vi "elevator_v1_working.vi"() -> ()   [LabVIEW 2020]
uses:
  State_enum.ctl
panel:
  in  "Stop Button":bool
  in  "1":bool
  in  "2":bool
  in  "3":bool
  out "Elevator":i8(slide) scale=0.0..10.0
  out "state":T1
  out "Destination floor":i32
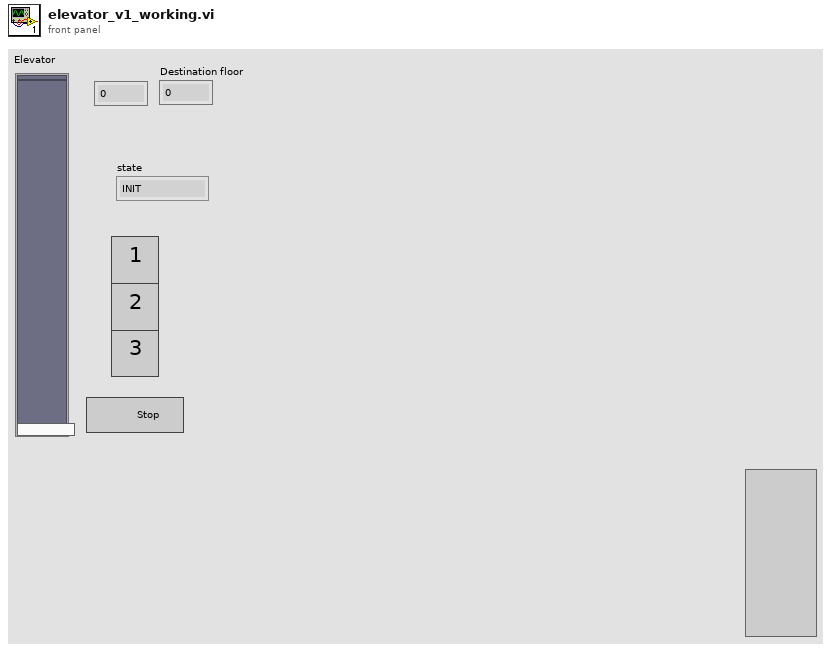
[diagram p1: front panel]
types:
  T1 = typedef "State_enum.ctl" = enum16{"INIT", "ATTENTE", "DEPLACEMENT", "PORTE_OUVERTE", "PORTE_FERMEE", "ARRET_URGENCE"}
  T2 = typedef "State_enum.ctl" = enum16{"Stopped", "Floor1", "Floor2", "Floor3"}
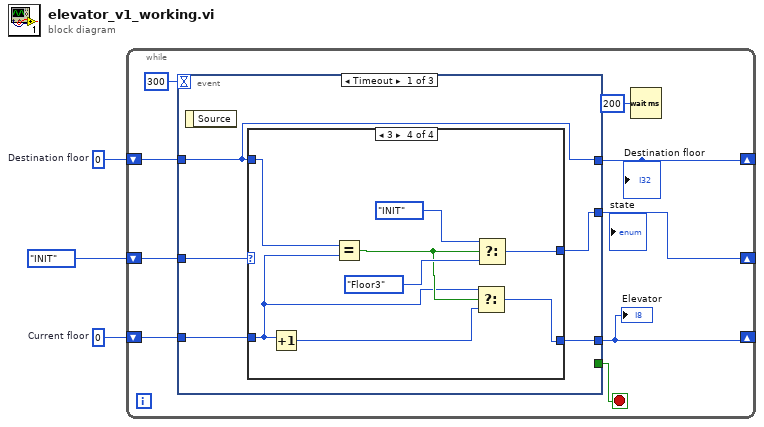
[diagram p0: block diagram]
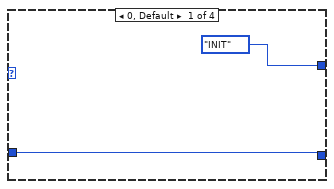
[diagram p2: hidden frame]
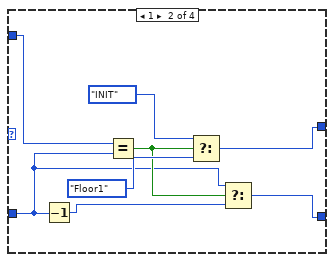
[diagram p3: hidden frame]
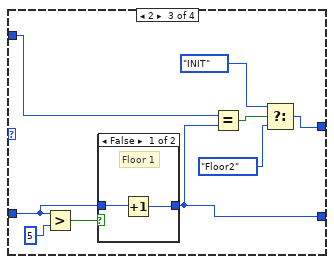
[diagram p4: hidden frame]
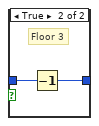
[diagram p5: hidden frame]
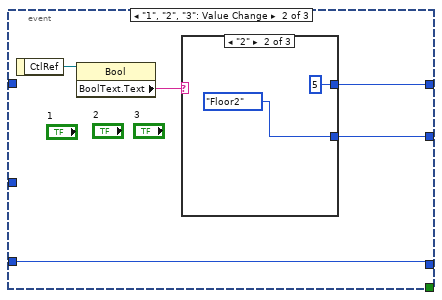
[diagram p6: hidden frame]
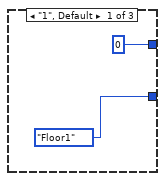
[diagram p7: hidden frame]
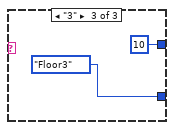
[diagram p8: hidden frame]
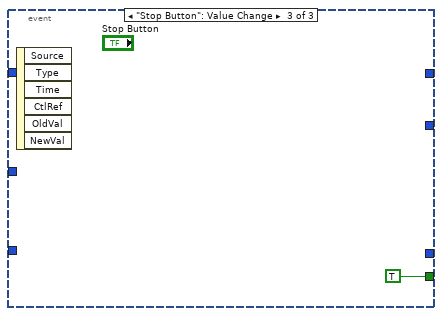
[diagram p9: hidden frame]
diagram:
  w2 = 0  # Current floor
  w3 = 0  # Destination floor
  n1 = while {
    shift-right: [w6] -> _
    shift-left: w3 -> [w7]
    shift-right: [w5] -> _
    shift-left: w2 -> [w9]
    shift-right: [w8] -> _
    shift-left: State_enum."INIT" ("state") -> [w10]
    stop <- w12 stop-if-true
    n2 = event shown="[0] Timeout" {
      selector: _ -> [_ _ _]
      dyn-events: _ -> [_ _ _]
      timeout: 300 -> [_ _ _]
      tunnel: [_ _ TRUE] -> w12
      tunnel: [w13 w51 _] -> w6
      tunnel: w10 -> [w17 _ _]
      tunnel: w9 -> [w16 w49 _]
      tunnel: [w15 w49 _] -> w5
      tunnel: [w14 w50 _] -> w8
      tunnel: w7 -> [w13 _ _]
      event Timeout {
        n3 = event-data() -> ()  [unwired: 1 in, 1 out]
        n4 = case shown="3" w17 {
          tunnel: w16 -> [w19 w22 w34 w42]
          tunnel: [w19 w20 w32 w41] -> w15
          tunnel: w13 -> [_ w27 w33 w48]
          tunnel: [State_enum."INIT" ("state") w26 w30 w47] -> w14
          frame 0, Default {
          }
          frame 1 {
            n5 = Decrement(x=w22) -> (x-1=w21:i32)
            n6 = Equal?(x=w27, y=w22) -> (x = y?=w23:bool)
            n7 = Select(t=State_enum."INIT" ("state"), s=w23, f=State_enum."Floor1" ("state")) -> (s? t:f=w26:u16)
            n8 = Select(t=w22, s=w23, f=w21) -> (s? t:f=w20:i32)
          }
          frame 2 {
            n9 = Greater?(x=w34, y=5 ("donde estamos")) -> (0:w35:bool)
            n10 = case shown="False" w35 {
              tunnel: w34 -> [w38 w40]
              tunnel: [w37 w39] -> w32
              frame False {
                # "Floor 1"
                n11 = Increment(x=w38) -> (x+1=w37:i32)
              }
              frame True {
                # "Floor 3"
                n12 = Decrement(x=w40) -> (x-1=w39:i32)
              }
            }
            n13 = Equal?(x=w33, y=w32) -> (x = y?=w31:bool)
            n14 = Select(t=State_enum."INIT" ("state"), s=w31, f=State_enum."Floor2" ("state")) -> (s? t:f=w30:u16)
          }
          frame 3 {
            n15 = Increment(x=w42) -> (x+1=w43:i32)
            n16 = Equal?(x=w48, y=w42) -> (x = y?=w44:bool)
            n17 = Select(t=w42, s=w44, f=w43) -> (s? t:f=w41:i32)
            n18 = Select(t=State_enum."INIT" ("state"), s=w44, f=State_enum."Floor3" ("state")) -> (s? t:f=w47:u16)
          }
        }
      }
      event "1", "2", "3": Value Change {
        n19 = event-data() -> ("CtlRef"=w53:refnum<vi>)  [unwired: 1 in]
        n20 = property class="Bool"(reference=w53) -> ("BoolText.Text"=w52:string)  [unwired: 1 in, 2 out]
        n21 = case shown="\"2\"" w52 {
          tunnel: [0 5 10] -> w51
          tunnel: [State_enum."Floor1" ("state") State_enum."Floor2" ("state") State_enum."Floor3" ("state")] -> w50
          frame "1", Default {
          }
          frame "2" {
          }
          frame "3" {
          }
        }
      }
      event "Stop Button": Value Change {
        n22 = event-data() -> ()  [unwired: 1 in, 6 out]
      }
    }
    "Elevator" <- w5
    "Destination floor" <- w6
    n23 = Wait (ms)(milliseconds to wait=u32 200) -> ()  [unwired: 1 out]
  }
